vi "Add Copyright to File.vi"(8 "error in (no error)":errorcluster, 10 "Copyright Text":string="© Company Name", 11 "File Path":path) -> (0 "error out":errorcluster)   [LabVIEW 2016, in "SLL Add Copyright.lvlib"]
doc: "Add/update copyright text to a LabVIEW file. Supported LabVIEW files are *.vi, *.ctl, *.lvlib, *.lvclass and *.lvproj."
uses:
  SLL Add Copyright.lvlib
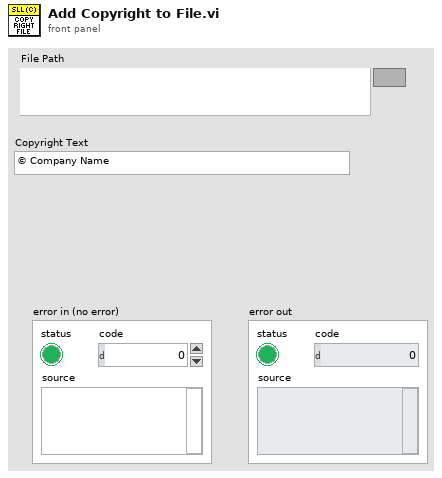
[diagram p1: front panel]
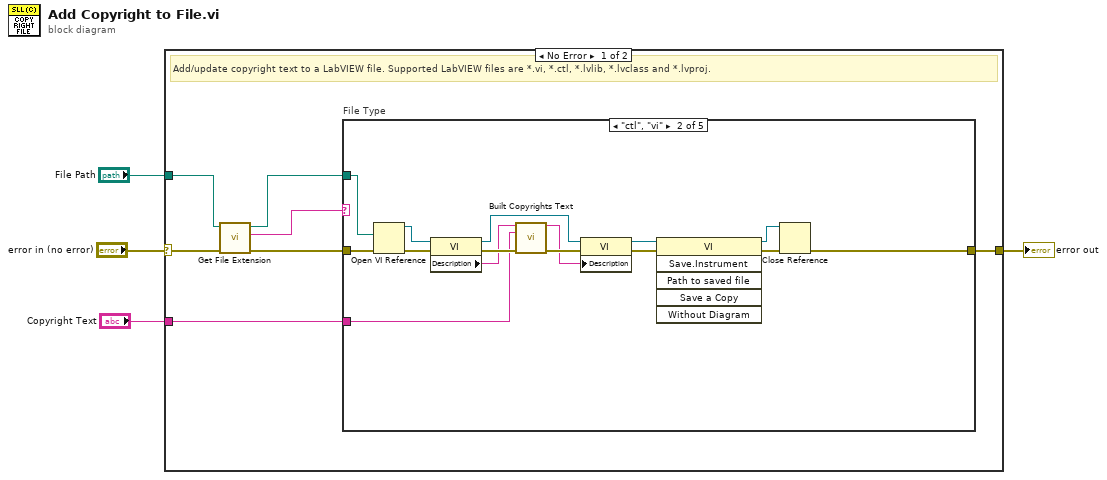
[diagram p0: block diagram]
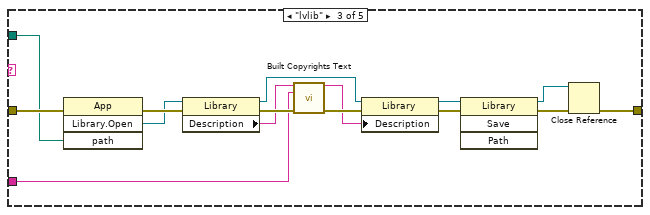
[diagram p3: hidden frame]
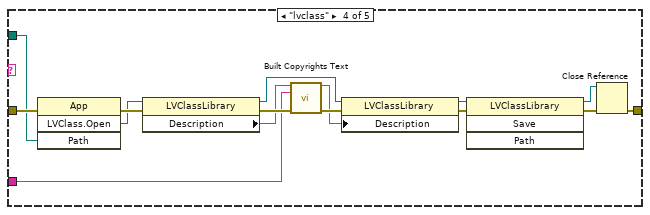
[diagram p4: hidden frame]
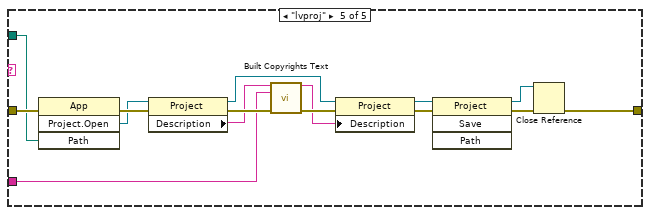
[diagram p5: hidden frame]
diagram:
  n1 = case shown="No Error" "error in (no error)" {
    selector: "error in (no error)" -> [w9 w73]
    tunnel: "Copyright Text" -> [w11 _]
    tunnel: [w10 w73] -> w3
    tunnel: "File Path" -> [w7 _]
    frame No Error {
      # "Add/update copyright text to a LabVIEW file. Supported LabVIEW files are *.vi, *.ctl, *.lvlib, *.lvclass and *.lvproj."
      n2 = call <vilib>:"Get File Extension.vi"("error in (no error)"=w9, "file"=w7) -> ("error out"=w8:errorcluster, "lowercase file extension"=w5:string, "dup file"=w6:path)  [unwired: 5 in, 2 out]
      n3 = case "File Type" shown="\"ctl\", \"vi\"" w5 {
        tunnel: [w12 w14 w29 w44 w59] -> w10
        tunnel: w8 -> [w12 w27 w42 w57 w72]
        tunnel: w6 -> [_ w25 w40 w55 w70]
        tunnel: w11 -> [_ w17 w36 w51 w66]
        frame Default {
        }
        frame "ctl", "vi" {
          n4 = Open VI Reference(vi path=w25, error in (no error)=w27) -> (vi reference=w24:refnum<vi>, error out=w26:errorcluster)  [unwired: 4 in]
          n5 = property class="VI"(reference=w24, error in=w26) -> (reference out=w19:refnum<vi>, error out=w23:errorcluster, "Description"=w21:string)
          n6 = call "Built Copyrights Text.vi"("Description in"=w21, "Licence Text"=w17, "error in"=w23) -> ("Description out"=w18:string, "error out"=w22:errorcluster)  [unwired: 11 in]
          n7 = property class="VI"(reference=w19, error in=w22, "Description"=w18) -> (reference out=w15:refnum<vi>, error out=w20:errorcluster)
          n8 = invoke class="VI" method="Save.Instrument"(reference=w15, error in=w20) -> (reference out=w13:refnum<vi>, error out=w16:errorcluster)  [unwired: 4 in, 4 out]
          n9 = Close Reference(reference=w13, error in (no error)=w16) -> (error out=w14:errorcluster)
        }
        frame "lvlib" {
          n10 = invoke class="App" method="Library.Open"(error in=w42, "path"=w40) -> (error out=w41:errorcluster, "Open Library"=w39:refnum<vi>)  [unwired: 2 in, 2 out]
          n11 = property class="Library"(reference=w39, error in=w41) -> (reference out=w32:refnum<vi>, error out=w38:errorcluster, "Description"=w37:string)
          n12 = call "Built Copyrights Text.vi"("Description in"=w37, "Licence Text"=w36, "error in"=w38) -> ("Description out"=w33:string, "error out"=w35:errorcluster)  [unwired: 11 in]
          n13 = property class="Library"(reference=w32, error in=w35, "Description"=w33) -> (reference out=w30:refnum<vi>, error out=w34:errorcluster)
          n14 = invoke class="Library" method="Save"(reference=w30, error in=w34) -> (reference out=w28:refnum<vi>, error out=w31:errorcluster)  [unwired: 2 in, 2 out]
          n15 = Close Reference(reference=w28, error in (no error)=w31) -> (error out=w29:errorcluster)
        }
        frame "lvclass" {
          n16 = invoke class="App" method="LVClass.Open"(error in=w57, "Path"=w55) -> (error out=w56:errorcluster, "LVClass.Open"=w54:refnum<vi>)  [unwired: 2 in, 2 out]
          n17 = property class="LVClassLibrary"(reference=w54, error in=w56) -> (reference out=w47:refnum<vi>, error out=w53:errorcluster, "Description"=w52:string)
          n18 = call "Built Copyrights Text.vi"("Description in"=w52, "Licence Text"=w51, "error in"=w53) -> ("Description out"=w48:string, "error out"=w50:errorcluster)  [unwired: 11 in]
          n19 = property class="LVClassLibrary"(reference=w47, error in=w50, "Description"=w48) -> (reference out=w45:refnum<vi>, error out=w49:errorcluster)
          n20 = invoke class="LVClassLibrary" method="Save"(reference=w45, error in=w49) -> (reference out=w43:refnum<vi>, error out=w46:errorcluster)  [unwired: 2 in, 2 out]
          n21 = Close Reference(reference=w43, error in (no error)=w46) -> (error out=w44:errorcluster)
        }
        frame "lvproj" {
          n22 = invoke class="App" method="Project.Open"(error in=w72, "Path"=w70) -> (error out=w71:errorcluster, "Project:Open"=w69:refnum<vi>)  [unwired: 2 in, 2 out]
          n23 = property class="Project"(reference=w69, error in=w71) -> (reference out=w62:refnum<vi>, error out=w68:errorcluster, "Description"=w67:string)
          n24 = call "Built Copyrights Text.vi"("Description in"=w67, "Licence Text"=w66, "error in"=w68) -> ("Description out"=w63:string, "error out"=w65:errorcluster)  [unwired: 11 in]
          n25 = property class="Project"(reference=w62, error in=w65, "Description"=w63) -> (reference out=w60:refnum<vi>, error out=w64:errorcluster)
          n26 = invoke class="Project" method="Save"(reference=w60, error in=w64) -> (reference out=w58:refnum<vi>, error out=w61:errorcluster)  [unwired: 2 in, 2 out]
          n27 = Close Reference(reference=w58, error in (no error)=w61) -> (error out=w59:errorcluster)
        }
      }
    }
    frame Error {
    }
  }
  "error out" <- w3
